vi "Test MQTT-7.1.2-1.vi"(8 "error in (no error)":errorcluster, 11 "Connection Config":refnum<class "Connection.lvclass">) -> (0 "error out":errorcluster, 3 "Connection Config dup":refnum<class "Connection.lvclass">)   [LabVIEW 2013]
uses:
  <vilib>/LabVIEW Open Source Project/MQTT Connection/MQTT_Connection/Connection/Connection.lvclass
  <vilib>/addons/_JKI Toolkits/Caraya/classes/Test/Test.lvclass
  <vilib>/LabVIEW Open Source Project/MQTT Client/Client class/Client.lvclass
  <vilib>/LabVIEW Open Source Project/MQTT Connection/MQTT_Base/Base Class/MQTT_Base.lvclass
  <vilib>/addons/_JKI Toolkits/Caraya/classes/Assert/Assert.lvclass
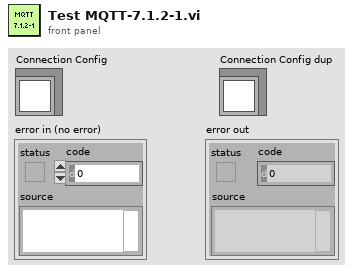
[diagram p1: front panel]
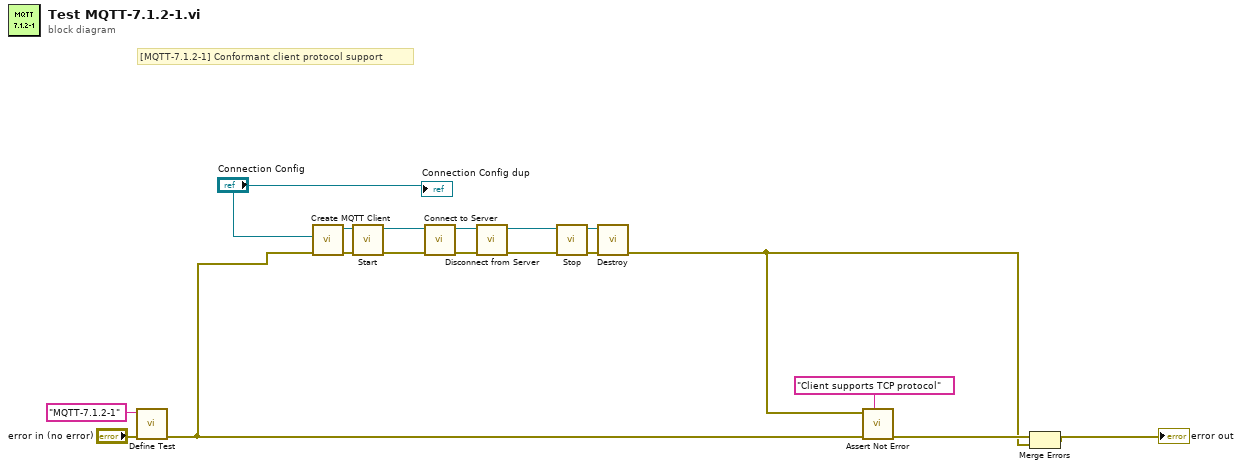
[diagram p0: block diagram]
diagram:
  # "[MQTT-7.1.2-1] Conformant client protocol support"
  n1 = call <vilib>:"Define Test.vi"("error in (no error)"="error in (no error)", "Label (VI Title)"="MQTT-7.1.2-1") -> ("error out"=w2:errorcluster)  [unwired: 9 in]
  n2 = call <vilib>:"Create MQTT Client.vi"("error in (no error)"=w2, "Connection Configuration"="Connection Config") -> ("error out"=w10:errorcluster, "Client out"=w11:refnum<class "Client.lvclass">)  [unwired: 8 in]
  n3 = call <vilib>:"Start.vi"("error in (no error)"=w10, "MQTT_Base in"=w11) -> ("error out"=w14:errorcluster, "MQTT_Base out"=w15:refnum<class "Client.lvclass">)  [unwired: 7 in, 1 out]
  n4 = call <vilib>:"Connect to Server.vi"("error in (no error)"=w14, "Client in"=w15) -> ("error out"=w4:errorcluster, "Client out"=w6:refnum<class "Client.lvclass">)  [unwired: 6 in, 2 out]
  n5 = call <vilib>:"Disconnect from Server.vi"("error in (no error)"=w4, "Client in"=w6) -> ("error out"=w3:errorcluster, "Client out"=w5:refnum<class "Client.lvclass">)  [unwired: 7 in, 1 out]
  n6 = call <vilib>:"Stop.vi"("error in (no error)"=w3, "MQTT_Base in"=w5) -> ("error out"=w12:errorcluster, "MQTT_Base out"=w13:refnum<class "Client.lvclass">)  [unwired: 7 in, 1 out]
  n7 = call <vilib>:"Destroy.vi"("error in (no error)"=w12, "MQTT_Base in"=w13) -> ("error out"=w8:errorcluster)  [unwired: 8 in, 1 out]
  n8 = call <vilib>:"Assert Not Error.vi"("Label"="Client supports TCP protocol", "error in (no error)"=w2, "Not Error?"=w8) -> ("error out"=w9:errorcluster)  [unwired: 8 in]
  n9 = Merge Errors(w9, w8) -> (→"error out":errorcluster)
  "Connection Config dup" <- "Connection Config"
